vi "Create Oneof Case Structure.vi"(8 "error in (no error)":errorcluster, 10 "Oneof Container Name":string, 11 "VI in":refnum<vi>) -> (0 "error out":errorcluster, 2 "CaseStructure out":refnum<vi>, 3 "VI out":refnum<vi>)   [LabVIEW 2019, in "gRPC Template Creation Utility.lvlib"]
uses:
  gRPC Template Creation Utility.lvlib
panel:
  # "Creates only a single frame with default case\nfor selected index of the oneof."
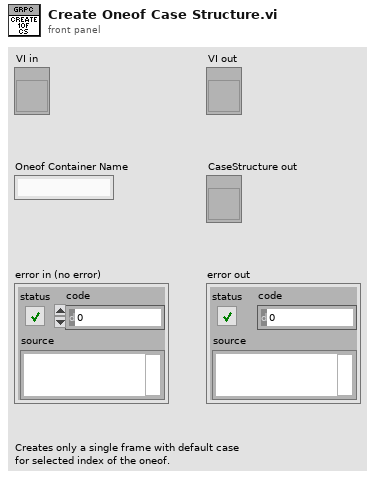
[diagram p1: front panel]
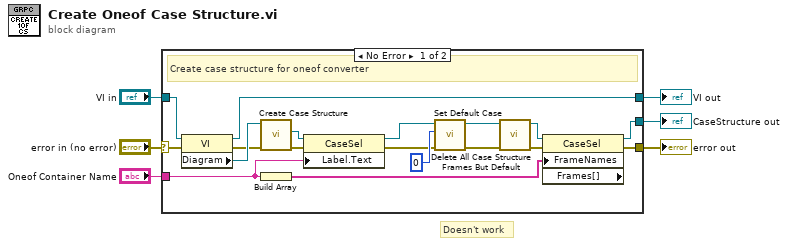
[diagram p0: block diagram]
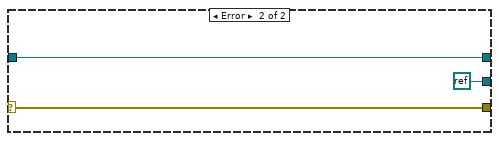
[diagram p2: hidden frame]
diagram:
  # "Doesn't work"
  n1 = case shown="No Error" "error in (no error)" {
    selector: "error in (no error)" -> [w23 w26]
    tunnel: "Oneof Container Name" -> [w9 _]
    tunnel: "VI in" -> [w24 w27]
    tunnel: [w7 w26] -> w3
    tunnel: [w13 w27] -> w2
    tunnel: [w11 refnum<k0> refnum] -> w1
    frame No Error {
      # "Create case structure for oneof converter"
      n2 = property class="VI"(reference=w24, error in=w23) -> (reference out=w13:refnum<vi>, error out=w21:errorcluster, "Diagram"=w22:refnum<vi>)
      n3 = call "Create Case Structure.vi"("error in (no error)"=w21, "Block Diagram in"=w22) -> ("error out"=w19:errorcluster, "Case Structure out"=w20:refnum<vi>)  [unwired: 7 in, 1 out]
      n4 = Build Array(w9) -> (w10:string[])
      n5 = property class="CaseSel"(reference=w20, error in=w19, "Label.Text"=w9) -> (reference out=w16:refnum<vi>, error out=w15:errorcluster)
      n6 = call "Set Default Case.vi"("error in (no error)"=w15, "Case Index"=0, "Case Structure in"=w16) -> ("error out"=w14:errorcluster, "Case Structure out"=w17:refnum<vi>)  [unwired: 7 in]
      n7 = call "Delete All Case Structure Frames But Default.vi"("error in (no error)"=w14, "CaseStructure in"=w17) -> ("error out"=w8:errorcluster, "CaseStructure out"=w12:refnum<vi>)  [unwired: 8 in]
      n8 = property class="CaseSel" props=["FrameNames", "Frames[]"](reference=w12, error in=w8, "FrameNames"=w10) -> (reference out=w11:refnum<vi>, error out=w7:errorcluster)  [unwired: 1 out]
    }
    frame Error {
    }
  }
  "error out" <- w3
  "VI out" <- w2
  "CaseStructure out" <- w1
